vi "set Sweep Type.vi"(8 "error in (no error)":errorcluster, 10 "Sweep Mode":T1, 11 "FSV-40N in":refnum<class "FSV-40N.lvclass">) -> (0 "error out":errorcluster, 3 "FSV-40N out":refnum<class "FSV-40N.lvclass">)   [LabVIEW 2023, in "Spectrum Analyzer.lvlib" / "FSV-40N.lvclass"]
uses:
  FSV-40N.lvclass
  FSV-40N.lvclass/FSV-40N.ctl
  TYPE DEFINITION/TYPE Sweep Type Select.ctl
  Spectrum Analyzer.lvlib
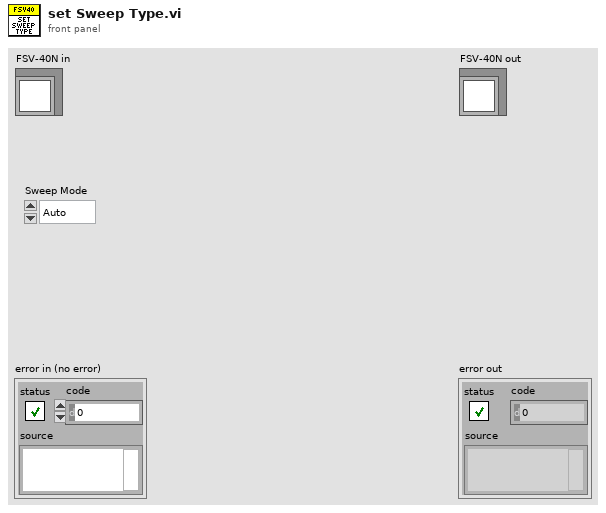
[diagram p1: front panel]
types:
  T1 = typedef "Spectrum Analyzer.lvlib/TYPE Sweep Type Select.ctl" = enum16{"Auto", "Sweep", "FFT"}
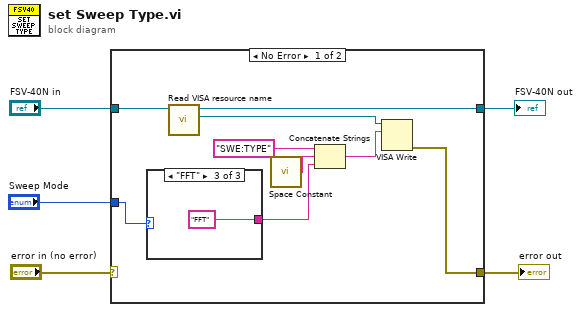
[diagram p0: block diagram]
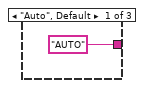
[diagram p2: hidden frame]
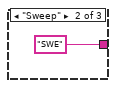
[diagram p3: hidden frame]
diagram:
  n1 = case shown="No Error" "error in (no error)" {
    selector: "error in (no error)" -> [_ w18]
    tunnel: "FSV-40N in" -> [w14 w19]
    tunnel: [w7 w19] -> w3
    tunnel: [w6 w18] -> w2
    tunnel: "Sweep Mode" -> [w13 _]
    frame No Error {
      n2 = case shown="\"FFT\"" w13 {
        tunnel: ["AUTO" "SWE" "FFT"] -> w10
        frame "Auto", Default {
        }
        frame "Sweep" {
        }
        frame "FFT" {
        }
      }
      n3 = call "Read VISA resource name.vi"("FSV-40N in"=w14) -> ("VISA resource name"=w9:refnum<visa-resource-name>, "FSV-40N out"=w7:refnum<class "FSV-40N.lvclass">)  [unwired: 8 in, 1 out]
      n4 = call <vilib>:"Space Constant.vi"() -> ("String"=w11:string)
      n5 = Concatenate Strings("SWE:TYPE" ("string"), w11, w10) -> (w8:string)
      n6 = VISA Write(VISA resource name=w9, write buffer=w8) -> (error out=w6:errorcluster)  [unwired: 1 in, 2 out]
    }
    frame Error {
    }
  }
  "error out" <- w2
  "FSV-40N out" <- w3
